vi "Draw_Machine.vi"(8 "Banner":string, 9 "Connected":bool, 10 "Y":bool[](array[boolean]), 11 "X":bool[](array[boolean])) -> (3 "Machine":picture)   [LabVIEW 2026]
doc: "Use this template to build a VI to use as a subVI."
panel:
  # "ÕfÃ÷£º®‹™CÌ¨ˆD¡£ß@Ì¨›]ÓÐÎ»ÖÃ»ØÊÚ£¬Ö»ÄÜÒÀ¸ÐœyÆ÷®‹Ç°‚È¡¢áá‚È¡¢ÖÐégÈý·N\nÎ»ÖÃ¡£"
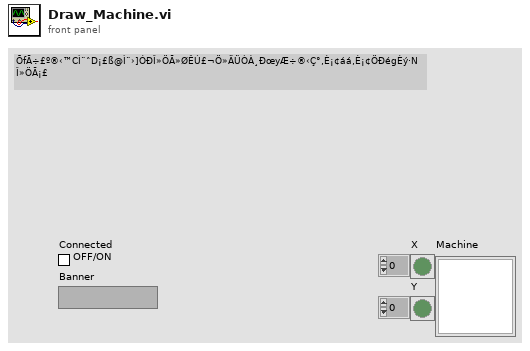
[diagram p1: front panel]
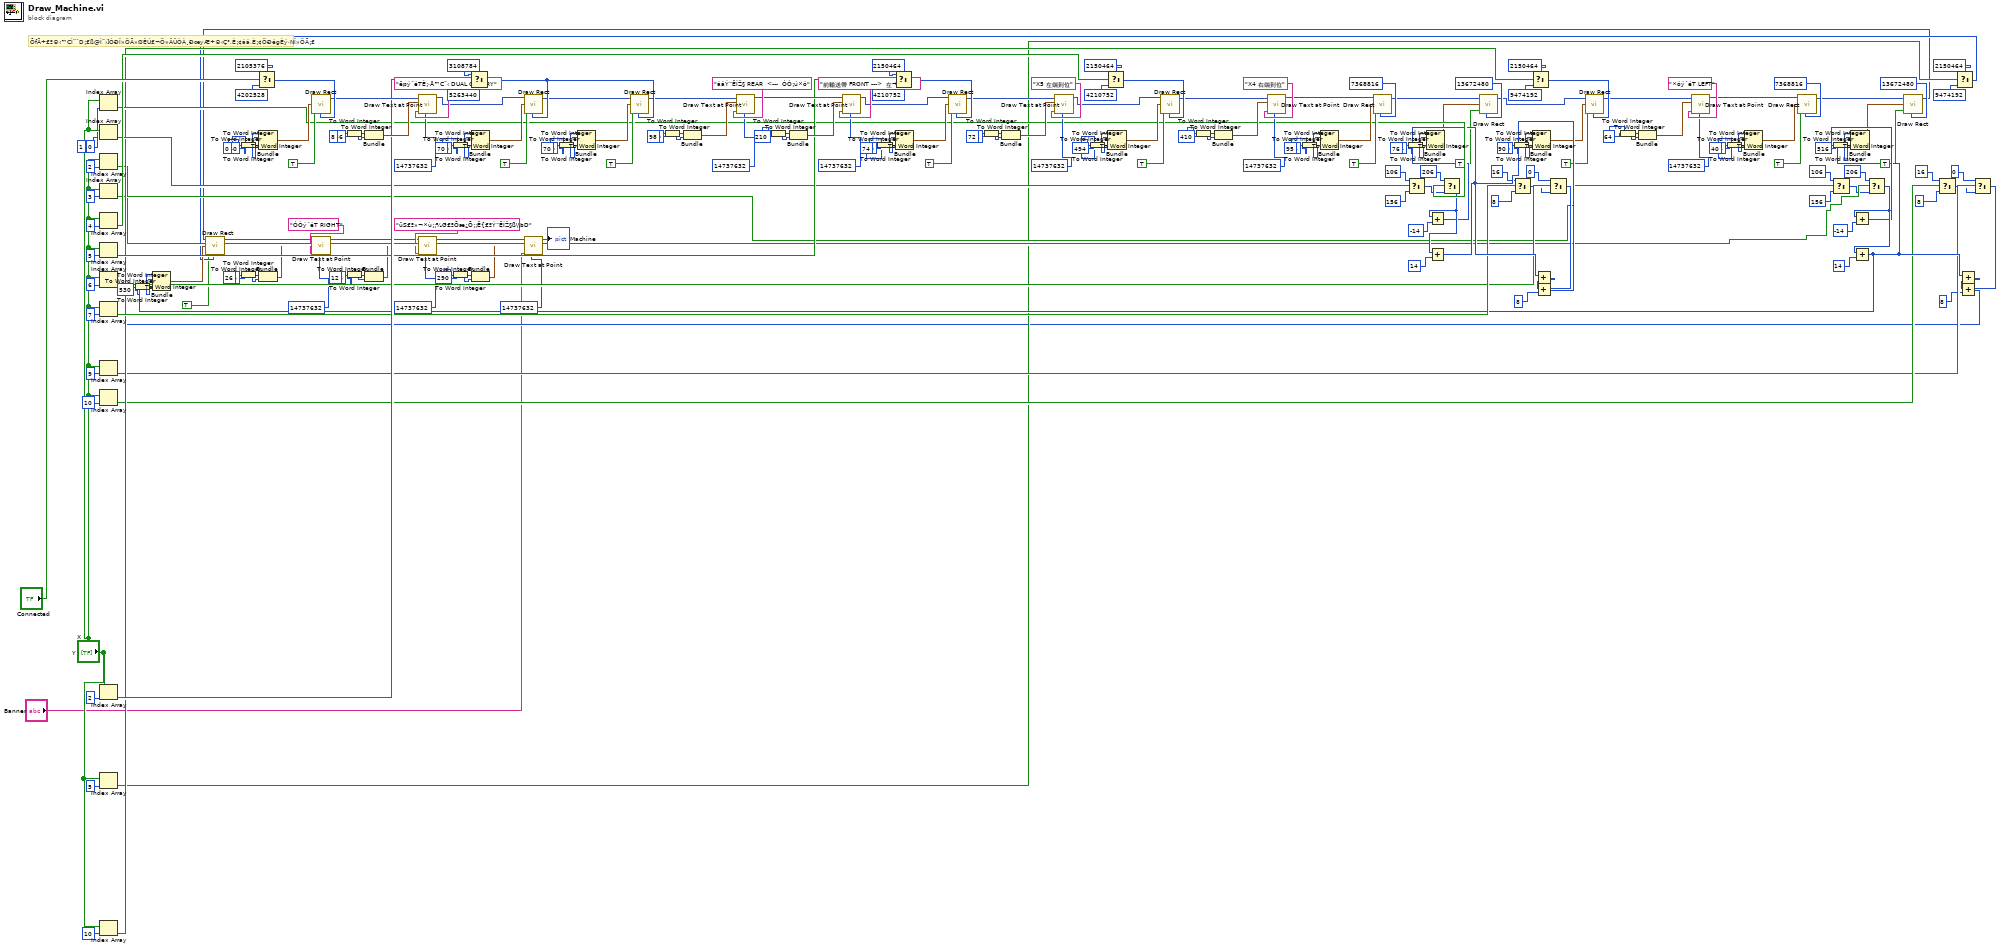
[diagram p0: block diagram]
diagram:
  # "ÕfÃ÷£º®‹™CÌ¨ˆD¡£ß@Ì¨›]ÓÐÎ»ÖÃ»ØÊÚ£¬Ö»ÄÜÒÀ¸ÐœyÆ÷®‹Ç°‚È¡¢áá‚È¡¢ÖÐégÈý·NÎ»ÖÃ¡£"
  n1 = Index Array(array="X", index=0) -> (element=w130:bool)
  n2 = Index Array(array="X", index=1) -> (element=w133:bool)
  n3 = Index Array(array="X", index=2) -> (element=w66:bool)
  n4 = Index Array(array="X", index=3) -> (element=w69:bool)
  n5 = Index Array(array="X", index=4) -> (element=w168:bool)
  n6 = Index Array(array="X", index=5) -> (element=w191:bool)
  n7 = Index Array(array="X", index=6) -> (element=w109:bool)
  n8 = Index Array(array="X", index=7) -> (element=w112:bool)
  n9 = Index Array(array="X", index=9) -> (element=w45:bool)
  n10 = Index Array(array="X", index=10) -> (element=w48:bool)
  n11 = Index Array(array="Y", index=2) -> (element=w233:bool)
  n12 = Index Array(array="Y", index=5) -> (element=w39:bool)
  n13 = Index Array(array="Y", index=10) -> (element=w103:bool)
  n14 = To Word Integer(number=550) -> (16bit integer=w32:i16)
  n15 = To Word Integer(number=530) -> (16bit integer=w35:i16)
  n16 = To Word Integer(number=290) -> (16bit integer=w245:i16)
  n17 = To Word Integer(number=640) -> (16bit integer=w247:i16)
  n18 = To Word Integer(number=0) -> (16bit integer=w249:i16)
  n19 = To Word Integer(number=0) -> (16bit integer=w251:i16)
  n20 = To Word Integer(number=26) -> (16bit integer=w22:i16)
  n21 = To Word Integer(number=504) -> (16bit integer=w24:i16)
  n22 = Select(t=2105376, s="Connected", f=4202528) -> (s? t:f=w243:i32)
  n23 = Bundle(w251, w249, w247, w245) -> (w244:cluster{i16, i16, i16, i16})  [unwired: 1 in]
  n24 = Bundle(w24, w22) -> (w21:cluster{i16, i16})  [unwired: 1 in]
  n25 = call <vilib>:"Draw Rect.vi"("rect"=w244, "fill?(F)"=TRUE, "color(black)"=w243) -> ("new picture"=w234:picture)  [unwired: 6 in]
  n26 = To Word Integer(number=8) -> (16bit integer=w238:i16)
  n27 = To Word Integer(number=236) -> (16bit integer=w240:i16)
  n28 = To Word Integer(number=268) -> (16bit integer=w14:i16)
  n29 = To Word Integer(number=12) -> (16bit integer=w16:i16)
  n30 = Bundle(w240, w238) -> (w237:cluster{i16, i16})  [unwired: 1 in]
  n31 = Bundle(w16, w14) -> (w13:cluster{i16, i16})  [unwired: 1 in]
  n32 = call <vilib>:"Draw Text at Point.vi"("text color(black)"=14737632, "text"="ëpýˆéTÈ¡·Å™C˜‹ DUAL GANTRY", "origin"=w237, "picture"=w234) -> ("new picture"=w219:picture)  [unwired: 6 in, 1 out]
  n33 = To Word Integer(number=122) -> (16bit integer=w223:i16)
  n34 = To Word Integer(number=570) -> (16bit integer=w225:i16)
  n35 = To Word Integer(number=90) -> (16bit integer=w227:i16)
  n36 = To Word Integer(number=70) -> (16bit integer=w229:i16)
  n37 = To Word Integer(number=268) -> (16bit integer=w6:i16)
  n38 = To Word Integer(number=290) -> (16bit integer=w8:i16)
  n39 = Select(t=3108784, s=w233, f=5263440) -> (s? t:f=w221:i32)
  n40 = Bundle(w229, w227, w225, w223) -> (w222:cluster{i16, i16, i16, i16})  [unwired: 1 in]
  n41 = Bundle(w8, w6) -> (w5:cluster{i16, i16})  [unwired: 1 in]
  n42 = call <vilib>:"Draw Rect.vi"("picture"=w219, "rect"=w222, "fill?(F)"=TRUE, "color(black)"=w221) -> ("new picture"=w208:picture)  [unwired: 5 in]
  n43 = To Word Integer(number=222) -> (16bit integer=w211:i16)
  n44 = To Word Integer(number=570) -> (16bit integer=w213:i16)
  n45 = To Word Integer(number=190) -> (16bit integer=w215:i16)
  n46 = To Word Integer(number=70) -> (16bit integer=w217:i16)
  n47 = Bundle(w217, w215, w213, w211) -> (w210:cluster{i16, i16, i16, i16})  [unwired: 1 in]
  n48 = call <vilib>:"Draw Rect.vi"("picture"=w208, "rect"=w210, "fill?(F)"=TRUE, "color(black)"=w221) -> ("new picture"=w200:picture)  [unwired: 5 in]
  n49 = To Word Integer(number=98) -> (16bit integer=w204:i16)
  n50 = To Word Integer(number=210) -> (16bit integer=w206:i16)
  n51 = Bundle(w206, w204) -> (w203:cluster{i16, i16})  [unwired: 1 in]
  n52 = call <vilib>:"Draw Text at Point.vi"("text color(black)"=14737632, "text"="ááÝ”ËÍŽ§ REAR  <---  ÓÒ¡ú×ó", "origin"=w203, "picture"=w200) -> ("new picture"=w192:picture)  [unwired: 6 in, 1 out]
  n53 = To Word Integer(number=198) -> (16bit integer=w196:i16)
  n54 = To Word Integer(number=210) -> (16bit integer=w198:i16)
  n55 = Bundle(w198, w196) -> (w195:cluster{i16, i16})  [unwired: 1 in]
  n56 = call <vilib>:"Draw Text at Point.vi"("text color(black)"=14737632, "text"="前輸送帶 FRONT --->  左→右", "origin"=w195, "picture"=w192) -> ("new picture"=w177:picture)  [unwired: 6 in, 1 out]
  n57 = To Word Integer(number=86) -> (16bit integer=w181:i16)
  n58 = To Word Integer(number=146) -> (16bit integer=w183:i16)
  n59 = To Word Integer(number=74) -> (16bit integer=w185:i16)
  n60 = To Word Integer(number=130) -> (16bit integer=w187:i16)
  n61 = Select(t=2150464, s=w191, f=4210752) -> (s? t:f=w179:i32)
  n62 = Bundle(w187, w185, w183, w181) -> (w180:cluster{i16, i16, i16, i16})  [unwired: 1 in]
  n63 = call <vilib>:"Draw Rect.vi"("picture"=w177, "rect"=w180, "fill?(F)"=TRUE, "color(black)"=w179) -> ("new picture"=w169:picture)  [unwired: 5 in]
  n64 = To Word Integer(number=72) -> (16bit integer=w173:i16)
  n65 = To Word Integer(number=152) -> (16bit integer=w175:i16)
  n66 = Bundle(w175, w173) -> (w172:cluster{i16, i16})  [unwired: 1 in]
  n67 = call <vilib>:"Draw Text at Point.vi"("text color(black)"=14737632, "text"="X5 左端到位", "origin"=w172, "picture"=w169) -> ("new picture"=w154:picture)  [unwired: 6 in, 1 out]
  n68 = To Word Integer(number=240) -> (16bit integer=w158:i16)
  n69 = To Word Integer(number=510) -> (16bit integer=w160:i16)
  n70 = To Word Integer(number=228) -> (16bit integer=w162:i16)
  n71 = To Word Integer(number=494) -> (16bit integer=w164:i16)
  n72 = Select(t=2150464, s=w168, f=4210752) -> (s? t:f=w156:i32)
  n73 = Bundle(w164, w162, w160, w158) -> (w157:cluster{i16, i16, i16, i16})  [unwired: 1 in]
  n74 = call <vilib>:"Draw Rect.vi"("picture"=w154, "rect"=w157, "fill?(F)"=TRUE, "color(black)"=w156) -> ("new picture"=w146:picture)  [unwired: 5 in]
  n75 = To Word Integer(number=244) -> (16bit integer=w150:i16)
  n76 = To Word Integer(number=410) -> (16bit integer=w152:i16)
  n77 = Bundle(w152, w150) -> (w149:cluster{i16, i16})  [unwired: 1 in]
  n78 = call <vilib>:"Draw Text at Point.vi"("text color(black)"=14737632, "text"="X4 右端到位", "origin"=w149, "picture"=w146) -> ("new picture"=w134:picture)  [unwired: 6 in, 1 out]
  n79 = To Word Integer(number=260) -> (16bit integer=w138:i16)
  n80 = To Word Integer(number=105) -> (16bit integer=w140:i16)
  n81 = To Word Integer(number=40) -> (16bit integer=w142:i16)
  n82 = To Word Integer(number=95) -> (16bit integer=w144:i16)
  n83 = Bundle(w144, w142, w140, w138) -> (w137:cluster{i16, i16, i16, i16})  [unwired: 1 in]
  n84 = call <vilib>:"Draw Rect.vi"("picture"=w134, "rect"=w137, "fill?(F)"=TRUE, "color(black)"=7368816) -> ("new picture"=w113:picture)  [unwired: 5 in]
  n85 = To Word Integer(number=124) -> (16bit integer=w119:i16)
  n86 = To Word Integer(number=76) -> (16bit integer=w123:i16)
  n87 = Select(t=106, s=w133, f=156) -> (s? t:f=w128:i32)
  n88 = Select(t=206, s=w130, f=w128) -> (s? t:f=w127:i32)
  n89 = Add(x=w127, y=-14) -> (x+y=w122:i32)
  n90 = To Word Integer(number=w122) -> (16bit integer=w121:i16)
  n91 = Add(x=w127, y=14) -> (x+y=w118:i32)
  n92 = To Word Integer(number=w118) -> (16bit integer=w117:i16)
  n93 = Bundle(w123, w121, w119, w117) -> (w116:cluster{i16, i16, i16, i16})  [unwired: 1 in]
  n94 = call <vilib>:"Draw Rect.vi"("picture"=w113, "rect"=w116, "fill?(F)"=TRUE, "color(black)"=13672480) -> ("new picture"=w90:picture)  [unwired: 5 in]
  n95 = To Word Integer(number=110) -> (16bit integer=w96:i16)
  n96 = To Word Integer(number=w118) -> (16bit integer=w98:i16)
  n97 = To Word Integer(number=90) -> (16bit integer=w99:i16)
  n98 = Select(t=16, s=w112, f=8) -> (s? t:f=w107:i32)
  n99 = Select(t=2150464, s=w103, f=9474192) -> (s? t:f=w92:i32)
  n100 = Select(t=0, s=w109, f=w107) -> (s? t:f=w106:i32)
  n101 = Add(x=w118, y=w106) -> (x+y=w105:i32)
  n102 = Add(x=w105, y=8) -> (x+y=w95:i32)
  n103 = To Word Integer(number=w95) -> (16bit integer=w94:i16)
  n104 = Bundle(w99, w98, w96, w94) -> (w93:cluster{i16, i16, i16, i16})  [unwired: 1 in]
  n105 = call <vilib>:"Draw Rect.vi"("picture"=w90, "rect"=w93, "fill?(F)"=TRUE, "color(black)"=w92) -> ("new picture"=w82:picture)  [unwired: 5 in]
  n106 = To Word Integer(number=26) -> (16bit integer=w86:i16)
  n107 = To Word Integer(number=64) -> (16bit integer=w88:i16)
  n108 = Bundle(w88, w86) -> (w85:cluster{i16, i16})  [unwired: 1 in]
  n109 = call <vilib>:"Draw Text at Point.vi"("text color(black)"=14737632, "text"="×óýˆéT LEFT", "origin"=w85, "picture"=w82) -> ("new picture"=w70:picture)  [unwired: 6 in, 1 out]
  n110 = To Word Integer(number=260) -> (16bit integer=w74:i16)
  n111 = To Word Integer(number=545) -> (16bit integer=w76:i16)
  n112 = To Word Integer(number=40) -> (16bit integer=w78:i16)
  n113 = To Word Integer(number=535) -> (16bit integer=w80:i16)
  n114 = Bundle(w80, w78, w76, w74) -> (w73:cluster{i16, i16, i16, i16})  [unwired: 1 in]
  n115 = call <vilib>:"Draw Rect.vi"("picture"=w70, "rect"=w73, "fill?(F)"=TRUE, "color(black)"=7368816) -> ("new picture"=w49:picture)  [unwired: 5 in]
  n116 = To Word Integer(number=564) -> (16bit integer=w55:i16)
  n117 = To Word Integer(number=516) -> (16bit integer=w59:i16)
  n118 = Select(t=106, s=w69, f=156) -> (s? t:f=w64:i32)
  n119 = Select(t=206, s=w66, f=w64) -> (s? t:f=w63:i32)
  n120 = Add(x=w63, y=-14) -> (x+y=w58:i32)
  n121 = To Word Integer(number=w58) -> (16bit integer=w57:i16)
  n122 = Add(x=w63, y=14) -> (x+y=w54:i32)
  n123 = To Word Integer(number=w54) -> (16bit integer=w34:i16)
  n124 = To Word Integer(number=w54) -> (16bit integer=w53:i16)
  n125 = Bundle(w59, w57, w55, w53) -> (w52:cluster{i16, i16, i16, i16})  [unwired: 1 in]
  n126 = call <vilib>:"Draw Rect.vi"("picture"=w49, "rect"=w52, "fill?(F)"=TRUE, "color(black)"=13672480) -> ("new picture"=w26:picture)  [unwired: 5 in]
  n127 = Select(t=16, s=w48, f=8) -> (s? t:f=w43:i32)
  n128 = Select(t=2150464, s=w39, f=9474192) -> (s? t:f=w28:i32)
  n129 = Select(t=0, s=w45, f=w43) -> (s? t:f=w42:i32)
  n130 = Add(x=w54, y=w42) -> (x+y=w41:i32)
  n131 = Add(x=w41, y=8) -> (x+y=w31:i32)
  n132 = To Word Integer(number=w31) -> (16bit integer=w30:i16)
  n133 = Bundle(w35, w34, w32, w30) -> (w29:cluster{i16, i16, i16, i16})  [unwired: 1 in]
  n134 = call <vilib>:"Draw Rect.vi"("picture"=w26, "rect"=w29, "fill?(F)"=TRUE, "color(black)"=w28) -> ("new picture"=w18:picture)  [unwired: 5 in]
  n135 = call <vilib>:"Draw Text at Point.vi"("text color(black)"=14737632, "text"="ÓÒýˆéT RIGHT", "origin"=w21, "picture"=w18) -> ("new picture"=w10:picture)  [unwired: 6 in, 1 out]
  n136 = call <vilib>:"Draw Text at Point.vi"("text color(black)"=14737632, "text"="üS£º»¬×ù¡¡¾G£ºÕæ¿Õ¡¡Ë{£ºÝ”ËÍŽ§ß\\ÞD", "origin"=w13, "picture"=w10) -> ("new picture"=w2:picture)  [unwired: 6 in, 1 out]
  n137 = call <vilib>:"Draw Text at Point.vi"("text color(black)"=14737632, "text"="Banner", "origin"=w5, "picture"=w2) -> ("new picture"=→"Machine":picture)  [unwired: 6 in, 1 out]
